vi "no-breakpoint.vi"() -> ()   [LabVIEW 2024]
panel:
  out "Numeric":i32
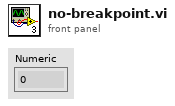
[diagram p1: front panel]
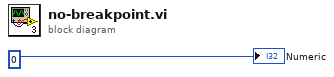
[diagram p0: block diagram]
diagram:
  "Numeric" <- 0
